vi "RunOperation.vi"(10 "Inputs":string[](array[string]), 11 "Test in":refnum<class "Test.lvclass">) -> (1 "Output/Failure":string, 2 "CLI Process Return Code":i32, 3 "Test out":refnum<class "Test.lvclass">)   [LabVIEW 2017, in "Test.lvclass"]
uses:
  Test.lvclass
  <vilib>/PNR/LVUnit/LVUnit Test Discoverer/LVUnit Test Discoverer.lvclass
  <vilib>/PNR/LVUnit/LVUnit Test Executor/LVUnit Test Executor.lvclass
  C:/Program Files (x86)/National Instruments/LabVIEW 2017/vi.lib/PNR/LVUnit/Test Executor/Test Executor.lvclass
  Test.lvclass/Test.ctl
  <vilib>/PNR/LVUnit/Cobertura/Project Inspector/Project Inspector.lvclass
  C:/Program Files (x86)/National Instruments/LabVIEW 2017/vi.lib/PNR/LVUnit/Cobertura/Project Inspector Base/Project Inspector Base.lvclass
  <vilib>/PNR/LVUnit/Cobertura/Code Inspector/Code Inspector.lvclass
  C:/Program Files (x86)/National Instruments/LabVIEW 2017/vi.lib/PNR/LVUnit/Cobertura/Code Inspector Base/Code Inspector Base.lvclass
  <vilib>/PNR/LVUnit/Test Executor/Test Executor.lvclass
  <vilib>/PNR/LVUnit/Code Coverage/Code Coverage.lvclass
  <vilib>/PNR/LVUnit/Cobertura/Cobertura.lvlib
  <vilib>/PNR/LVUnit/JUnit/JUnit.lvlib
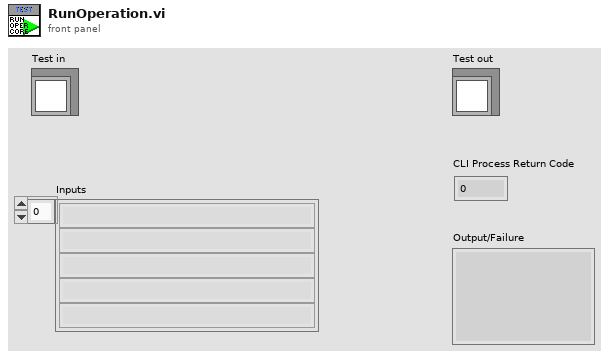
[diagram p1: front panel]
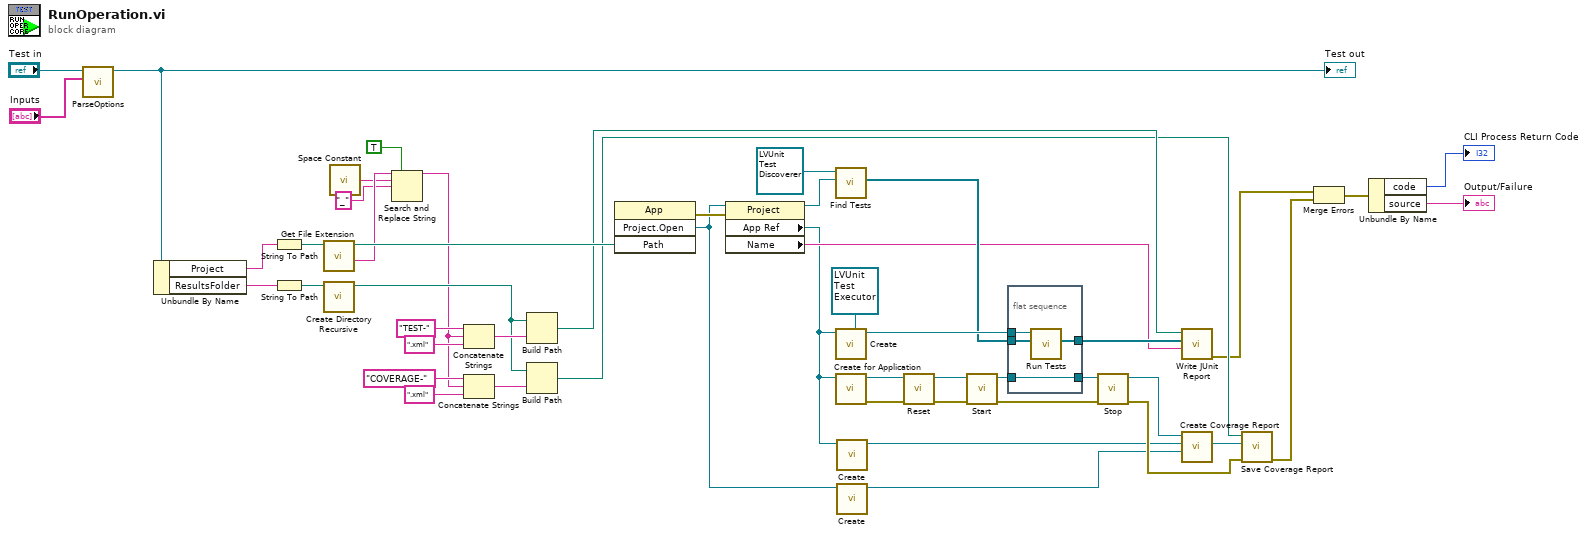
[diagram p0: block diagram]
diagram:
  n1 = call "ParseOptions.vi"("Options"="Inputs", "Test in"="Test in") -> ("Test out"=w45:refnum<class "Test.lvclass">)  [unwired: 8 in, 1 out]
  "Test out" <- w45
  n2 = Unbundle By Name(w45) -> ("Project"=w44:string, "ResultsFolder"=w42:string)
  n3 = String To Path(string=w44) -> (path=w40:path)
  n4 = String To Path(string=w42) -> (path=w41:path)
  n5 = call <vilib>:"Get File Extension.vi"("file"=w40) -> ("filename without extension"=w12:string, "dup file"=w36:path)  [unwired: 6 in, 3 out]
  n6 = call <vilib>:"Create Directory Recursive.vi"("directory"=w41) -> ("directory copy"=w22:path)  [unwired: 4 in, 2 out]
  n7 = call <vilib>:"Space Constant.vi"() -> ("String"=w11:string)
  n8 = Search and Replace String(replace all?=TRUE ("replace all? (F)"), input string=w12, search string=w11, replace string="_") -> (result string=w8:string)  [unwired: 4 in, 3 out]
  n9 = Concatenate Strings("TEST-" ("string"), w8, ".xml" ("string")) -> (w37:string)
  n10 = Concatenate Strings("COVERAGE-" ("string"), w8, ".xml" ("string")) -> (w23:string)
  n11 = Build Path(base path=w22, name or relative path=w37) -> (appended path=w26:path)
  n12 = Build Path(base path=w22, name or relative path=w23) -> (appended path=w20:path)
  n13 = invoke class="App" method="Project.Open"("Path"=w36) -> (error out=w43:errorcluster, "Project:Open"=w2:refnum<vi>)  [unwired: 3 in, 2 out]
  n14 = property class="Project"(reference=w2, error in=w43) -> (reference out=w33:refnum<vi>, "App Ref"=w4:refnum<vi>, "Name"=w13:string)  [unwired: 1 out]
  n15 = call-dynamic "Find Tests.vi"("Project Refnum"=w33, "LVUnit Test Discoverer in"=refnum<class "LVUnit Test Discoverer.lvclass"> refnum ("LVUnit Test Discoverer")) -> ("Test Cases"=w29:refnum<class "Test Case.lvclass">[])  [unwired: 7 in, 2 out]
  n16 = call <vilib>:"Create.vi"("Test Executor in"=refnum<class "LVUnit Test Executor.lvclass"> refnum ("LVUnit Test Executor"), "Application"=w4) -> ("Test Executor"=w30:refnum<class "LVUnit Test Executor.lvclass">)  [unwired: 8 in, 1 out]
  n17 = call <vilib>:"Create for Application.vi"("Application"=w4) -> ("error out"=w14:errorcluster, "CodeCoverage out"=w31:refnum<class "Code Coverage.lvclass">)  [unwired: 9 in]
  n18 = call <vilib>:"Create.vi"("Application"=w4) -> ("Code Inspector"=w3:refnum<class "Code Inspector.lvclass">)  [unwired: 9 in, 1 out]
  n19 = call <vilib>:"Create.vi"("Project"=w2) -> ("Project Inspector"=w1:refnum<class "Project Inspector.lvclass">)  [unwired: 9 in, 1 out]
  n20 = call <vilib>:"Reset.vi"("error in (no error)"=w14, "CodeCoverage in"=w31) -> ("error out"=w7:errorcluster, "CodeCoverage out"=w32:refnum<class "Code Coverage.lvclass">)  [unwired: 8 in]
  n21 = call <vilib>:"Start.vi"("error in (no error)"=w7, "CodeCoverage in"=w32) -> ("error out"=w15:errorcluster, "CodeCoverage out"=w6:refnum<class "Code Coverage.lvclass">)  [unwired: 8 in]
  n22 = flat-sequence {
    tunnel: w30 -> [w53]
    tunnel: w29 -> [w52]
    tunnel: [w51] -> w27
    tunnel: w6 -> [w50]
    tunnel: [w50] -> w5
    frame #0 {
      n23 = call-dynamic "Run Tests.vi"("Test Cases"=w52, "LVUnit Test Executor in"=w53) -> ("Test Results"=w51:refnum<class "Test Result.lvclass">[])  [unwired: 7 in, 2 out]
    }
  }
  n24 = call <vilib>:"Stop.vi"("error in (no error)"=w15, "CodeCoverage in"=w5) -> ("error out"=w16:errorcluster, "CodeCoverage out"=w28:refnum<class "Code Coverage.lvclass">)  [unwired: 8 in]
  n25 = call <vilib>:"Write JUnit Report.vi"("Project Name"=w13, "Test Results"=w27, "File Path"=w26) -> ("error out"=w18:errorcluster)  [unwired: 8 in]
  n26 = call <vilib>:"Create Coverage Report.vi"("Project Inspector"=w1, "Code Inspector"=w3, "CodeCoverage in"=w28) -> ("Coverage"=w21:refnum<class "Coverage.lvclass">)  [unwired: 7 in, 1 out]
  n27 = call <vilib>:"Save Coverage Report.vi"("error in (no error)"=w16, "Coverage"=w21, "Path"=w20) -> ("error out"=w17:errorcluster)  [unwired: 8 in]
  n28 = Merge Errors(w18, w17) -> (w19:errorcluster)
  n29 = Unbundle By Name(w19) -> ("code"=→"CLI Process Return Code":i32, "source"=→"Output/Failure":string)
